vi "RenameClass.vi"(0 "ClassWriterNative.lvclass":refnum<class "ClassWriterNative.lvclass">, 1 "ClassRef":refnum<vi>, 2 "NewClassPath":path, 4 "RelinkWholeProject":bool, 5 "error in (no error)":errorcluster) -> (14 "ClassWriterNative.lvclass":refnum<class "ClassWriterNative.lvclass">, 19 "error out":errorcluster={"status"=TRUE, "code"=1026, "source"="Invoke Node in ClassWriterGOOP300.lvclass:RenameClass.vi"})   [LabVIEW 2020, in "ClassWriterNative.lvclass"]
uses:
  ClassWriterNative.lvclass
  f5b91c3c-2b4b-4460-aca0-bdbd4ce9a051.vi
  313d9ab2-2167-4cbd-8752-784b5e159654.vi
  a4843f61-b178-4b78-a5e8-dfb32b4ec01f.vi
  Common/ScriptingFunctions/Scripting.lvclass
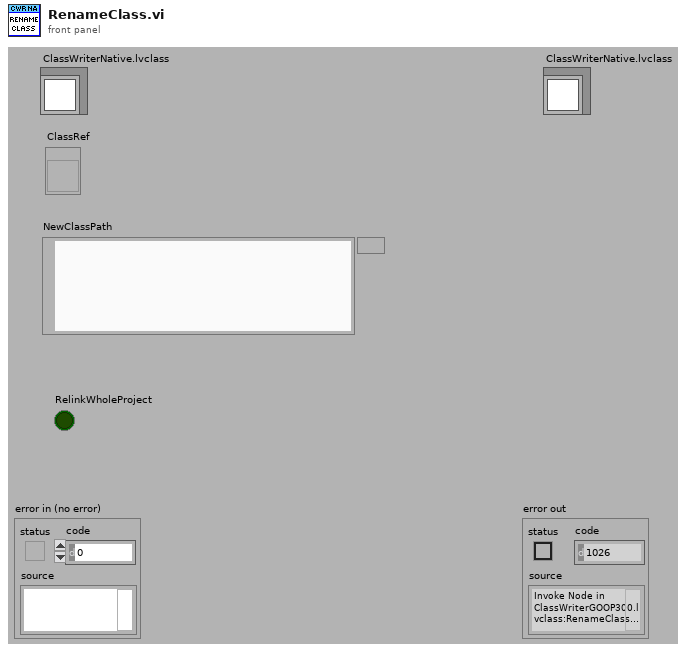
[diagram p1: front panel]
types:
  T1 = cluster{"SubClass":bool, "ClassFiles":path[], "ClassName":string, "ClassFolder":path, "VIs":refnum<vi>[], "TemplateFolder":path, "ViSubDirs":string[], "TemplateName":string, "BaseClassFolder":path, "TemplateClasses":refnum<vi>[], "Application":refnum<vi>}
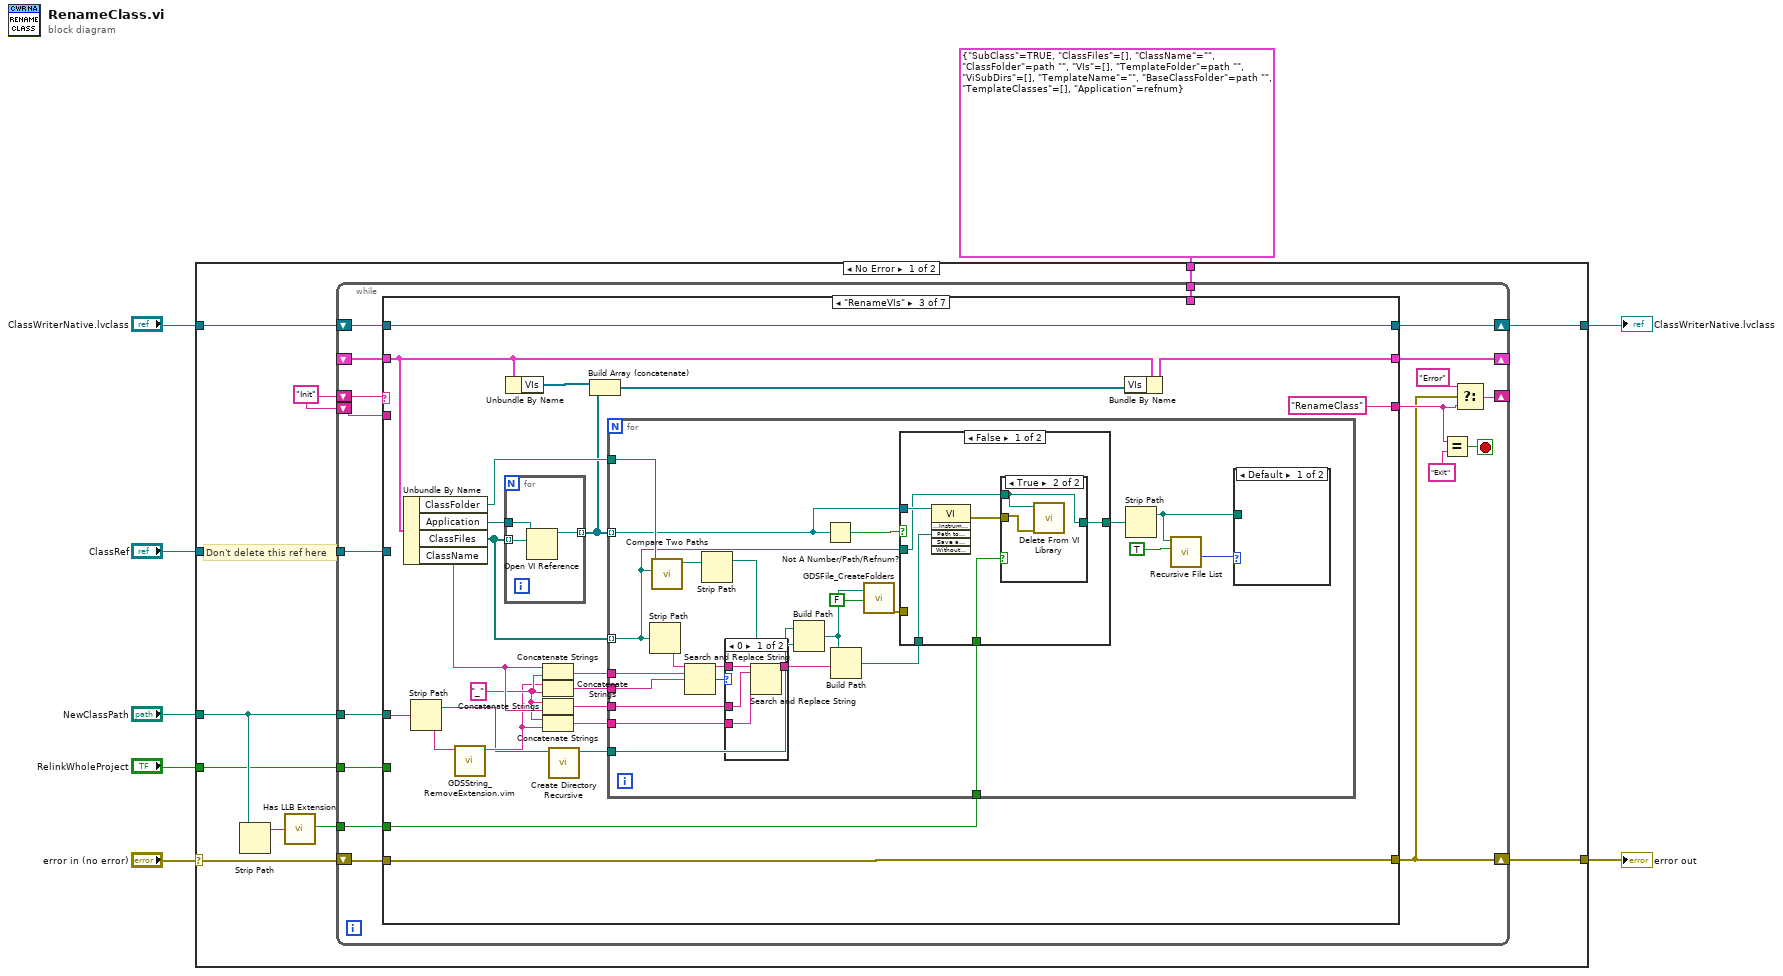
[diagram p0: block diagram]
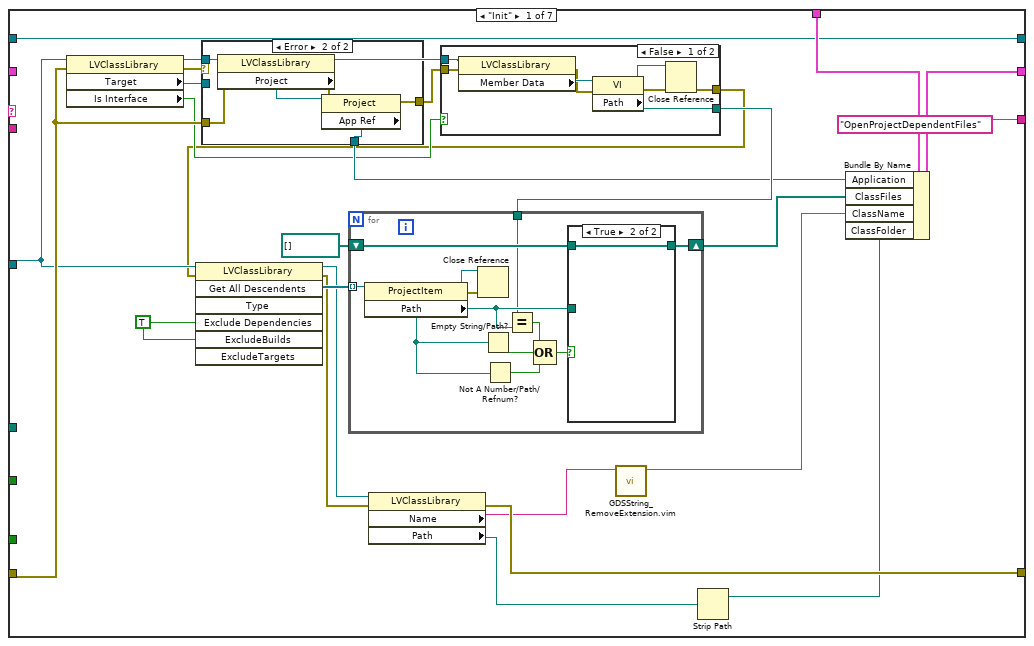
[diagram p2: hidden frame]
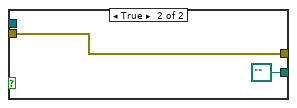
[diagram p3: hidden frame]
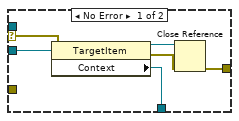
[diagram p4: hidden frame]
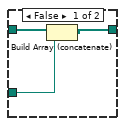
[diagram p5: hidden frame]
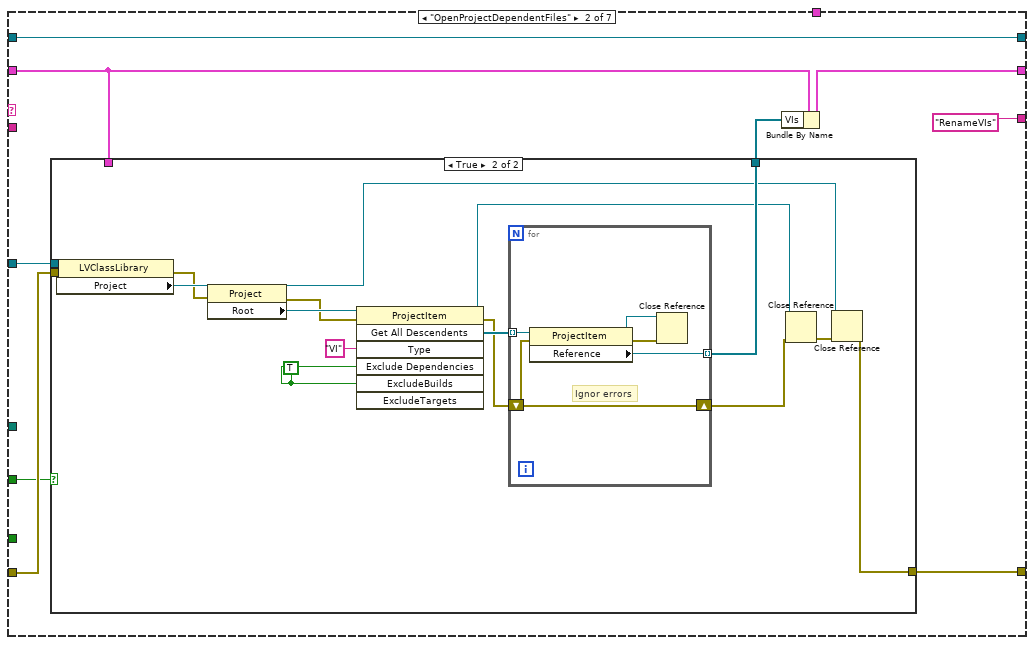
[diagram p6: hidden frame]
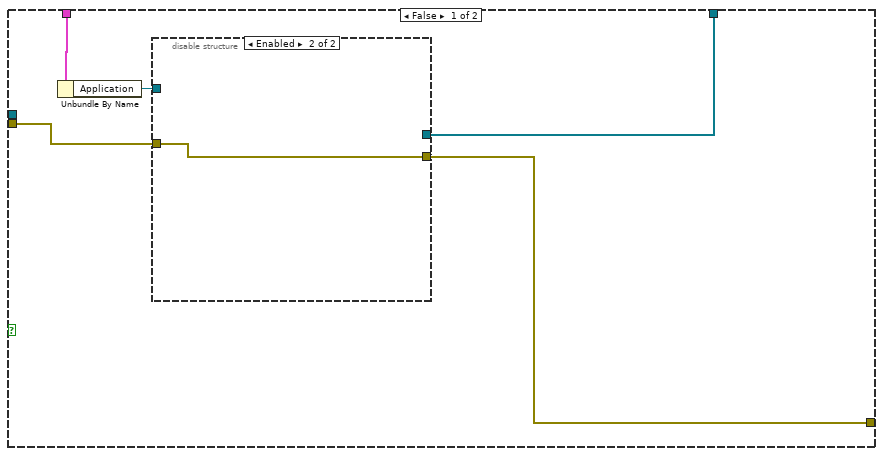
[diagram p7: hidden frame]
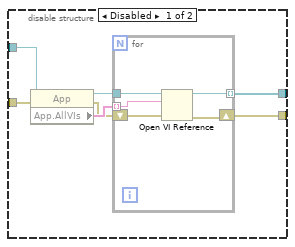
[diagram p8: hidden frame]
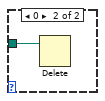
[diagram p10: hidden frame]
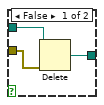
[diagram p11: hidden frame]
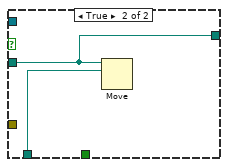
[diagram p12: hidden frame]
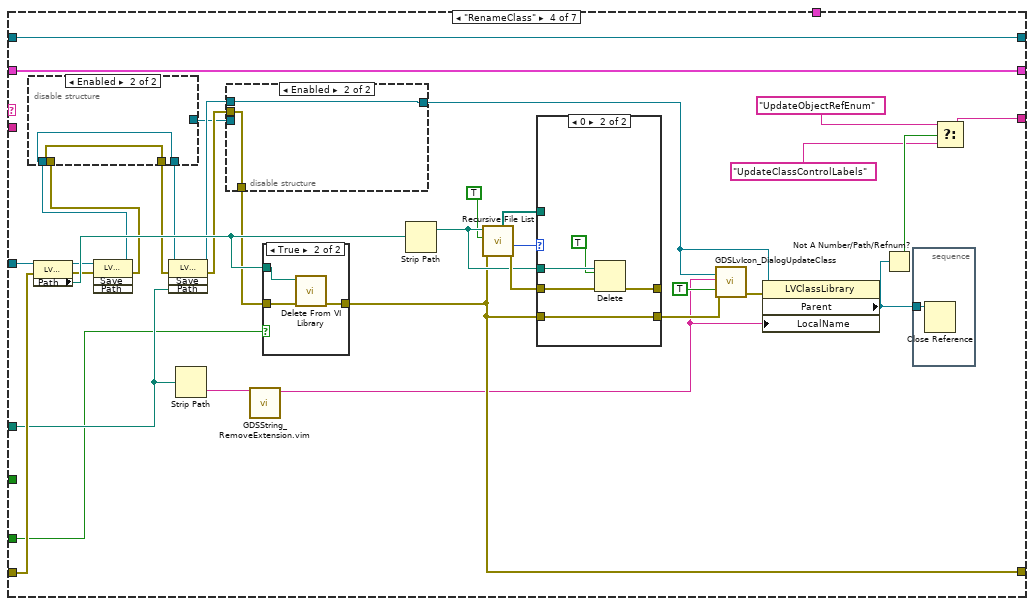
[diagram p13: hidden frame]
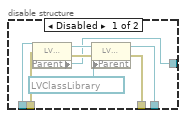
[diagram p14: hidden frame]
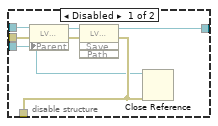
[diagram p15: hidden frame]
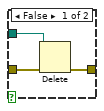
[diagram p16: hidden frame]
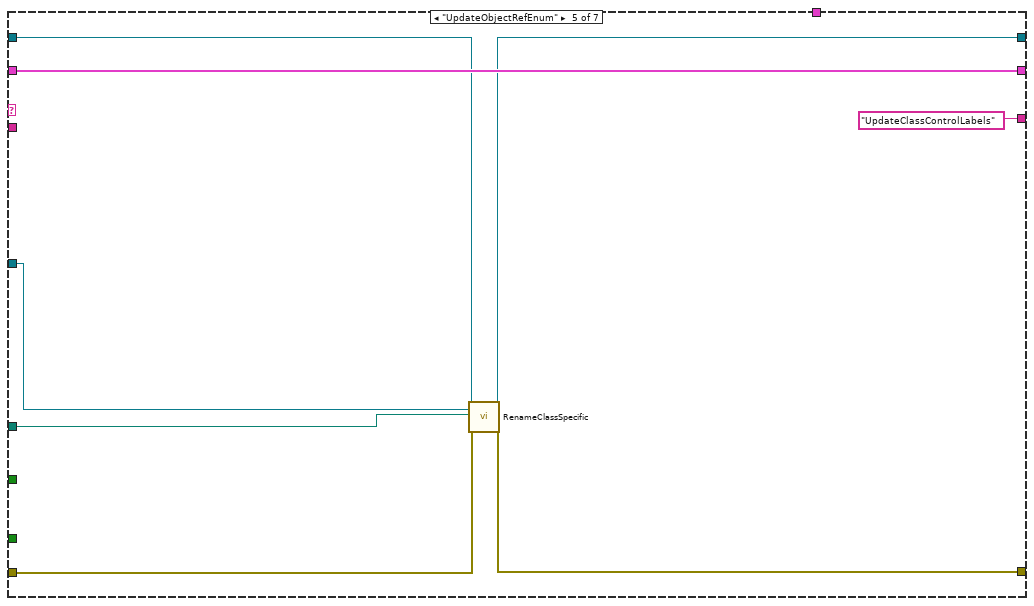
[diagram p18: hidden frame]
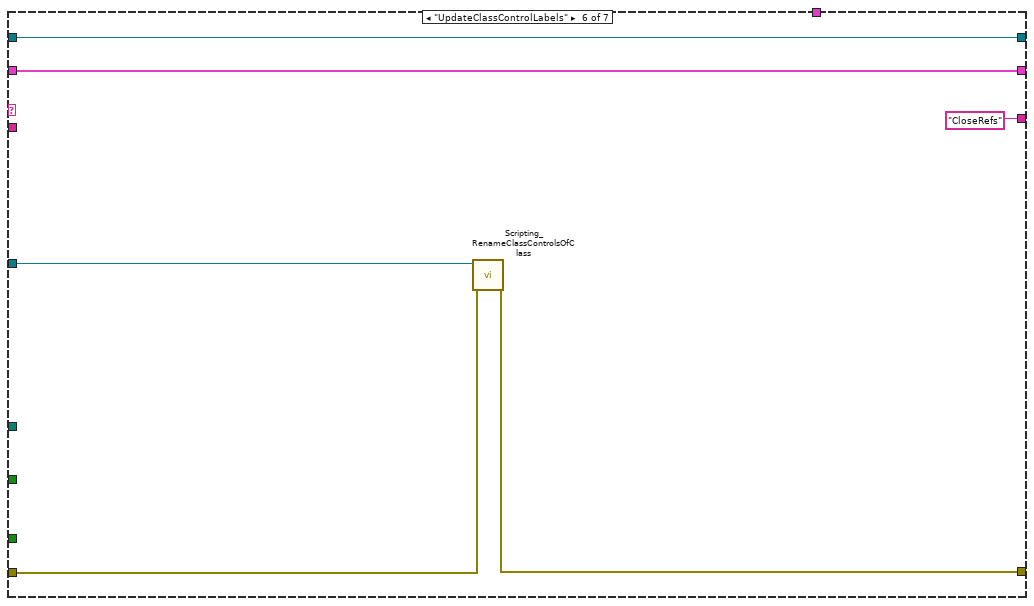
[diagram p19: hidden frame]
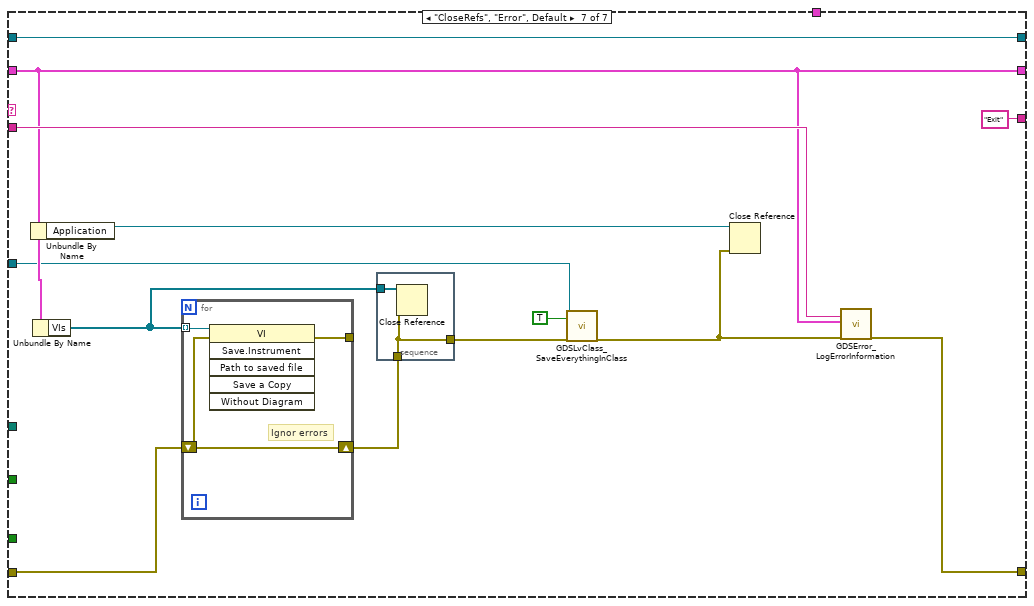
[diagram p20: hidden frame]
diagram:
  n1 = case shown="No Error" "error in (no error)" {
    selector: "error in (no error)" -> [w18 w317]
    tunnel: [w17 w317] -> w8
    tunnel: "ClassRef" -> [w19 _]
    tunnel: T1 {"SubClass"=TRUE, "ClassFiles"=[], "ClassName"="", "ClassFolder"=path "", "VIs"=[], "TemplateFolder"=path "", "ViSubDirs"=[], "TemplateName"="", "BaseClassFolder"=path "", "TemplateClasses"=[], "Application"=refnum} ("output cluster") -> [w16 _]
    tunnel: "NewClassPath" -> [w12 _]
    tunnel: "ClassWriterNative.lvclass" -> [w14 w316]
    tunnel: [w13 w316] -> w2
    tunnel: "RelinkWholeProject" -> [w9 _]
    frame No Error {
      w15 = "Init"
      # "Don't delete this ref here"
      n2 = Strip Path(path=w12) -> (stripped path=w10:path)  [unwired: 1 out]
      n3 = call <vilib>:"Has LLB Extension.vi"("path"=w10) -> ("path to VI library?"=w11:bool)
      n4 = while {
        tunnel: w19 -> [w37]
        shift-right: [w26] -> w17
        shift-left: w18 -> [w36]
        shift-right: [w31] -> _
        shift-left: w15 -> [w27]
        shift-right: [w34] -> _
        shift-left: _ -> [w35]
        tunnel: w16 -> [w29]
        tunnel: w12 -> [w25]
        shift-left: w15 -> [w24]
        shift-right: [w22] -> w13
        shift-left: w14 -> [w23]
        tunnel: w11 -> [w21]
        tunnel: w9 -> [w20]
        stop <- w32 stop-if-true
        n5 = case shown="\"RenameVIs\"" w27 {
          tunnel: w35 -> [_ w100 w163 w250 w290 w296 w305]
          tunnel: [w61 w105 w164 w250 w290 w296 w305] -> w34
          tunnel: w37 -> [w44 w107 _ w249 w289 w292 w302]
          tunnel: w36 -> [w45 w106 w169 w248 w287 w294 w309]
          tunnel: [w54 w103 w169 w220 w286 w293 w307] -> w26
          tunnel: ["OpenProjectDependentFiles" "RenameVIs" "RenameClass" w242 "UpdateClassControlLabels" "CloseRefs" "Exit"] -> w28
          tunnel: w29 -> [w60 _ _ _ _ _ _]
          tunnel: w25 -> [_ _ w167 w246 w288 _ _]
          tunnel: w24 -> [_ _ _ _ _ _ w306]
          tunnel: w23 -> [w48 w102 w158 w239 w285 w295 w304]
          tunnel: [w48 w102 w158 w239 w284 w295 w304] -> w22
          tunnel: w21 -> [_ _ w152 w232 _ _ _]
          tunnel: w20 -> [_ w101 _ _ _ _ _]
          frame "Init" {
            w47 = TRUE ("ExcludeDependencies")
            n6 = property class="LVClassLibrary"(reference=w44, error in=w45) -> (reference out=w38:refnum<vi>, error out=w46:errorcluster, "Target"=w50:refnum<vi>, "Is Interface"=w43:bool)
            n7 = case shown="Error" w46 {
              selector: w46 -> [w73 _]
              tunnel: w50 -> [w78 _]
              tunnel: [w75 w81] -> w42
              tunnel: [w74 w82] -> w49
              tunnel: w38 -> [_ w84]
              tunnel: w45 -> [_ w79]
              frame No Error {
                n8 = property class="TargetItem"(reference=w78, error in=w73) -> (reference out=w76:refnum<vi>, error out=w77:errorcluster, "Context"=w74:refnum<vi>)
                n9 = Close Reference(reference=w76, error in (no error)=w77) -> (error out=w75:errorcluster)
              }
              frame Error {
                n10 = property class="LVClassLibrary"(reference=w84, error in=w79) -> (error out=w80:errorcluster, "Project"=w83:refnum<vi>)  [unwired: 1 out]
                n11 = property class="Project"(reference=w83, error in=w80) -> (error out=w81:errorcluster, "App Ref"=w82:refnum<vi>)  [unwired: 1 out]
              }
            }
            n12 = case shown="False" w43 {
              tunnel: [w68 path "" ("Path")] -> w51
              tunnel: w42 -> [w66 w72]
              tunnel: [w64 w72] -> w41
              tunnel: w38 -> [w63 _]
              frame False {
                n13 = property class="LVClassLibrary"(reference=w63, error in=w66) -> (error out=w65:errorcluster, "Member Data"=w67:refnum<vi>)  [unwired: 1 out]
                n14 = property class="VI"(reference=w67, error in=w65) -> (reference out=w69:refnum<vi>, error out=w70:errorcluster, "Path"=w68:path)
                n15 = Close Reference(reference=w69, error in (no error)=w70) -> (error out=w64:errorcluster)
              }
              frame True {
              }
            }
            n16 = invoke class="LVClassLibrary" method="Get All Descendents"(reference=w44, error in=w41, "Exclude Dependencies"=w47, "ExcludeBuilds"=w47) -> (reference out=w56:refnum<vi>, error out=w55:errorcluster, "All Descendents"=w59:refnum<vi>[])  [unwired: 3 in, 4 out]
            n17 = for {
              tunnel: w59 -> [w91] mode=indexing
              shift-right: [w94] -> w57
              shift-left: path[] [] -> [w95]
              tunnel: w51 -> [w89]
              n18 = property class="ProjectItem"(reference=w91) -> (reference out=w93:refnum<vi>, error out=w92:errorcluster, "Path"=w90:path)  [unwired: 1 in]
              n19 = Close Reference(reference=w93, error in (no error)=w92) -> ()  [unwired: 1 out]
              n20 = Empty String/Path?(string/path=w90) -> (empty?=w87:bool)
              n21 = Not A Number/Path/Refnum?(number/path/refnum=w90) -> (NaN/Path/Refnum?=w88:bool)
              n22 = Equal?(x=w89, y=w90) -> (x = y?=w86:bool)
              n23 = Compound Arithmetic op=OR(w86, w87, w88) -> (w85:bool)
              n24 = case shown="True" w85 {
                tunnel: w95 -> [w98 w99]
                tunnel: w90 -> [w97 _]
                tunnel: [w96 w99] -> w94
                frame False {
                  n25 = Build Array (concatenate)(w98, w97) -> (w96:path[])
                }
                frame True {
                }
              }
            }
            n26 = property class="LVClassLibrary"(reference=w56, error in=w55) -> (error out=w54:errorcluster, "Name"=w40:string, "Path"=w53:path)  [unwired: 1 out]
            n27 = call "GDSString_RemoveExtension.vim"("NameWithExtension"=w40) -> ("NameWithoutExtension"=w39:string)  [unwired: 9 in, 1 out]
            n28 = Strip Path(path=w53) -> (stripped path=w52:path)  [unwired: 1 out]
            n29 = Bundle By Name(cluster=w60, "Application"=w49, "ClassFiles"=w57, "ClassName"=w39, "ClassFolder"=w52) -> (w61:T1)
          }
          frame "OpenProjectDependentFiles" {
            n30 = case shown="True" w101 {
              tunnel: w107 -> [_ w142]
              tunnel: w106 -> [w109 w137]
              tunnel: [w113 w134] -> w104
              tunnel: [w112 w128] -> w103
              tunnel: w100 -> [w111 _]
              frame False {
                n31 = Unbundle By Name(w111) -> ("Application"=w110:refnum<vi>)
                n32 = disable-structure shown="Enabled" {
                  disable-tunnel: [w117 _] -> w113
                  disable-tunnel: [w116 w126] -> w112
                  disable-tunnel: w110 -> [w115 _]
                  disable-tunnel: w109 -> [w114 w126]
                  frame Disabled {
                    n33 = property class="App"(reference=w115, error in=w114) -> (reference out=w120:refnum<vi>, error out=w118:errorcluster, "App.AllVIs"=w119:string[])
                    n34 = for {
                      tunnel: w120 -> [w125]
                      tunnel: w119 -> [w124] mode=indexing
                      shift-right: [w122] -> w116
                      shift-left: w118 -> [w123]
                      tunnel: [w121] -> w117 mode=indexing
                      n35 = Open VI Reference(application reference (local)=w125, vi path=w124, error in (no error)=w123) -> (vi reference=w121:refnum<vi>, error out=w122:errorcluster)  [unwired: 3 in]
                    }
                  }
                  frame Enabled {
                  }
                }
              }
              frame True {
                w127 = TRUE ("ExcludeDependencies")
                n36 = property class="LVClassLibrary"(reference=w142, error in=w137) -> (error out=w138:errorcluster, "Project"=w141:refnum<vi>)  [unwired: 1 out]
                n37 = property class="Project"(reference=w141, error in=w138) -> (reference out=w129:refnum<vi>, error out=w136:errorcluster, "Root"=w140:refnum<vi>)
                n38 = invoke class="ProjectItem" method="Get All Descendents"(reference=w140, error in=w136, "Type"="VI", "Exclude Dependencies"=w127, "ExcludeBuilds"=w127) -> (reference out=w131:refnum<vi>, error out=w133:errorcluster, "All Descendents"=w135:refnum<vi>[])  [unwired: 2 in, 4 out]
                n39 = for {
                  tunnel: w135 -> [w147] mode=indexing
                  tunnel: [w146] -> w134 mode=indexing
                  shift-right: [w143] -> w132
                  shift-left: w133 -> [w143]
                  # "Ignor errors"
                  n40 = property class="ProjectItem"(reference=w147, error in=w143) -> (reference out=w144:refnum<vi>, error out=w145:errorcluster, "Reference"=w146:refnum<vi>)
                  n41 = Close Reference(reference=w144, error in (no error)=w145) -> ()  [unwired: 1 out]
                }
                n42 = Close Reference(reference=w131, error in (no error)=w132) -> (error out=w130:errorcluster)
                n43 = Close Reference(reference=w129, error in (no error)=w130) -> (error out=w128:errorcluster)
              }
            }
            n44 = Bundle By Name(cluster=w100, "VIs"=w104) -> (w105:T1)
          }
          frame "RenameVIs" {
            w155 = "_" ("string")
            n45 = Unbundle By Name(w163) -> ("ClassFolder"=w165:path, "Application"=w159:refnum<vi>, "ClassFiles"=w168:path[], "ClassName"=w156:string)
            n46 = Strip Path(path=w167) -> (stripped path=w148:path, name=w151:string)
            n47 = call "GDSString_RemoveExtension.vim"("NameWithExtension"=w151) -> ("NameWithoutExtension"=w150:string)  [unwired: 9 in, 1 out]
            n48 = for {
              tunnel: w168 -> [w216] mode=indexing
              tunnel: [w215] -> w161 mode=indexing
              tunnel: w159 -> [w214]
              n49 = Open VI Reference(application reference (local)=w214, vi path=w216) -> (vi reference=w215:refnum<vi>)  [unwired: 4 in, 1 out]
            }
            n50 = Unbundle By Name(w163) -> ("VIs"=w162:refnum<vi>[])
            n51 = Concatenate Strings(w156, w155) -> (w157:string)
            n52 = Concatenate Strings(w150, w155) -> (w166:string)
            n53 = Concatenate Strings(w155, w156) -> (w154:string)
            n54 = Concatenate Strings(w155, w150) -> (w153:string)
            n55 = call <vilib>:"Create Directory Recursive.vi"("directory"=w148) -> ("directory copy"=w149:path)  [unwired: 4 in, 2 out]
            n56 = Build Array (concatenate)(w162, w161) -> (w160:refnum<vi>[])
            n57 = for {
              tunnel: w161 -> [w180] mode=indexing
              tunnel: w168 -> [w183] mode=indexing
              tunnel: w157 -> [w194]
              tunnel: w166 -> [w193]
              tunnel: w149 -> [w192]
              tunnel: w165 -> [w191]
              tunnel: w154 -> [w177]
              tunnel: w153 -> [w176]
              tunnel: w152 -> [w175]
              n58 = Strip Path(path=w183) -> (name=w190:string)  [unwired: 1 out]
              n59 = call <vilib>:"Compare Two Paths.vi"("Path 2"=w183, "Path 1"=w191) -> ("Relative Path from 1 to 2"=w189:path)  [unwired: 6 in, 3 out]
              n60 = Search and Replace String(input string=w190, search string=w194, replace string=w193) -> (result string=w179:string, number of replacements=w171:i32)  [unwired: 5 in, 2 out]
              n61 = Strip Path(path=w189) -> (stripped path=w188:path)  [unwired: 1 out]
              n62 = case shown="0" w171 {
                tunnel: w179 -> [w198 w199]
                tunnel: [w197 w199] -> w178
                tunnel: w177 -> [w196 _]
                tunnel: w176 -> [w195 _]
                frame 0 {
                  n63 = Search and Replace String(input string=w198, search string=w196, replace string=w195) -> (result string=w197:string)  [unwired: 5 in, 3 out]
                }
                frame Default {
                }
              }
              n64 = Build Path(base path=w192, name or relative path=w188) -> (appended path=w187:path)
              n65 = Not A Number/Path/Refnum?(number/path/refnum=w180) -> (NaN/Path/Refnum?=w185:bool)
              n66 = Build Path(base path=w187, name or relative path=w178) -> (appended path=w182:path)
              n67 = call "GDSFile_CreateFolders.vi"("Path"=w187, "Promt if folder\ndoes not exists?"=FALSE ("Promt if folder\ndoes not exists?")) -> ("error out"=w184:errorcluster)  [unwired: 13 in, 4 out]
              n68 = case shown="False" w185 {
                tunnel: w184 -> [_ _]
                tunnel: w183 -> [w202 w212]
                tunnel: w182 -> [w205 w213]
                tunnel: [w204 w212] -> w181
                tunnel: w180 -> [w206 _]
                tunnel: w175 -> [w201 _]
                frame False {
                  n69 = invoke class="VI" method="Save.Instrument"(reference=w206, "Path to saved file"=w205) -> (error out=w203:errorcluster)  [unwired: 4 in, 5 out]
                  n70 = case shown="True" w201 {
                    tunnel: [w209 w211] -> w204
                    tunnel: w203 -> [w208 w210]
                    tunnel: w202 -> [w207 w211]
                    frame False {
                      n71 = Delete(path (use dialog)=w207, error in=w208) -> (deleted path=w209:path)  [unwired: 3 in, 2 out]
                    }
                    frame True {
                      n72 = call <vilib>:"Delete From VI Library.vi"("error in (no error)"=w210, "path"=w211) -> ()  [unwired: 9 in, 1 out]
                    }
                  }
                }
                frame True {
                  n73 = Move(source path=w212, 10:w213) -> ()  [unwired: 3 in, 3 out]
                }
              }
              n74 = Strip Path(path=w181) -> (stripped path=w173:path)  [unwired: 1 out]
              n75 = call <vilib>:"Recursive File List.vi"("Treat LLBs as Folders?"=TRUE, "Folder Path"=w173) -> ("Number of Files"=w172:i32)  [unwired: 5 in, 4 out]
              n76 = case shown="Default" w172 {
                tunnel: w173 -> [_ w200]
                frame Default {
                }
                frame 0 {
                  n77 = Delete(path (use dialog)=w200) -> ()  [unwired: 4 in, 3 out]
                }
              }
            }
            n78 = Bundle By Name(cluster=w163, "VIs"=w160) -> (w164:T1)
          }
          frame "RenameClass" {
            n79 = property class="LVClassLibrary"(reference=w249, error in=w248) -> (reference out=w231:refnum<vi>, error out=w230:errorcluster, "Path"=w233:path)
            n80 = invoke class="LVClassLibrary" method="Save"(reference=w231, error in=w230) -> (reference out=w229:refnum<vi>, error out=w228:errorcluster)  [unwired: 2 in, 2 out]
            n81 = disable-structure shown="Enabled" {
              disable-tunnel: w229 -> [w258 w260]
              disable-tunnel: w228 -> [w257 w259]
              disable-tunnel: [w253 w260] -> w227
              disable-tunnel: [w252 w259] -> w226
              disable-tunnel: [w251 _] -> w217
              frame Disabled {
                n82 = property class="LVClassLibrary"(reference=w258, error in=w257) -> (reference out=w256:refnum<vi>, error out=w255:errorcluster, "Parent"=w251:refnum<vi>)
                n83 = property class="LVClassLibrary"(reference=w256, error in=w255, "Parent"=refnum<vi> refnum ("Parent Class")) -> (reference out=w253:refnum<vi>, error out=w252:errorcluster)
              }
              frame Enabled {
              }
            }
            n84 = invoke class="LVClassLibrary" method="Save"(reference=w227, error in=w226, "Path"=w246) -> (reference out=w225:refnum<vi>, error out=w224:errorcluster)  [unwired: 1 in, 2 out]
            n85 = Strip Path(path=w246) -> (name=w219:string)  [unwired: 1 out]
            n86 = disable-structure shown="Enabled" {
              disable-tunnel: w225 -> [w267 w268]
              disable-tunnel: w224 -> [w266 w269]
              disable-tunnel: [w263 w268] -> w223
              disable-tunnel: [w262 w269] -> w222
              disable-tunnel: w217 -> [w261 _]
              frame Disabled {
                n87 = property class="LVClassLibrary"(reference=w267, error in=w266, "Parent"=w261) -> (reference out=w265:refnum<vi>, error out=w264:errorcluster)
                n88 = invoke class="LVClassLibrary" method="Save"(reference=w265, error in=w264) -> (reference out=w263:refnum<vi>, error out=w262:errorcluster)  [unwired: 2 in, 2 out]
                n89 = Close Reference(reference=w261, error in (no error)=w262) -> ()  [unwired: 1 out]
              }
              frame Enabled {
              }
            }
            n90 = call "GDSString_RemoveExtension.vim"("NameWithExtension"=w219) -> ("NameWithoutExtension"=w218:string)  [unwired: 9 in, 1 out]
            n91 = case shown="True" w232 {
              tunnel: w222 -> [w272 w273]
              tunnel: w233 -> [w271 w275]
              tunnel: [w270 w274] -> w220
              frame False {
                n92 = Delete(path (use dialog)=w271, error in=w272) -> (error out=w270:errorcluster)  [unwired: 3 in, 2 out]
              }
              frame True {
                n93 = call <vilib>:"Delete From VI Library.vi"("error in (no error)"=w273, "path"=w275) -> ("error out"=w274:errorcluster)  [unwired: 9 in]
              }
            }
            n94 = Strip Path(path=w233) -> (stripped path=w235:path)  [unwired: 1 out]
            n95 = call <vilib>:"Recursive File List.vi"("error in (no error)"=w220, "Treat LLBs as Folders?"=TRUE, "Folder Path"=w235) -> ("error out"=w237:errorcluster, "Number of Files"=w238:i32, "All Folders"=w236:path[])  [unwired: 4 in, 2 out]
            n96 = case shown="0" w238 {
              tunnel: w235 -> [_ w283]
              tunnel: w237 -> [w278 w280]
              tunnel: [w278 w281] -> _
              tunnel: w236 -> [_ _]
              tunnel: [w277 w279] -> w221
              tunnel: w220 -> [w277 w279]
              frame Default {
              }
              frame 0 {
                n97 = Delete(path (use dialog)=w283, entire hierarchy (F)=TRUE, error in=w280) -> (error out=w281:errorcluster)  [unwired: 2 in, 2 out]
              }
            }
            n98 = call "GDSLvIcon_DialogUpdateClass.vi"("ClassPath(FilePath/ProjectTreePath/LvCLassRef)"=w223, "ClassName"=w218, "AutoUpdate"=TRUE, "error in (no error)"=w221) -> ("error out"=w245:errorcluster)  [unwired: 12 in, 3 out]
            n99 = property class="LVClassLibrary"(reference=w223, error in=w245, "LocalName"=w218) -> ("Parent"=w244:refnum<vi>)  [unwired: 2 out]
            n100 = Not A Number/Path/Refnum?(number/path/refnum=w244) -> (NaN/Path/Refnum?=w243:bool)
            n101 = stacked-sequence {
              tunnel: w244 -> [w276]
              frame #0 {
                n102 = Close Reference(reference=w276) -> ()  [unwired: 1 in, 1 out]
              }
            }
            n103 = Select(t="UpdateObjectRefEnum", s=w243, f="UpdateClassControlLabels") -> (s? t:f=w242:string)
          }
          frame "UpdateObjectRefEnum" {
            n104 = call-dynamic "RenameClassSpecific.vi"("ClassWriterNative.lvclass"=w285, "ClassRef"=w289, "NewClassPath"=w288, "error in"=w287) -> ("ClassWriterNative.lvclass"=w284:refnum<class "ClassWriterNative.lvclass">, "error out"=w286:errorcluster)  [unwired: 14 in]
          }
          frame "UpdateClassControlLabels" {
            n105 = call "Scripting_RenameClassControlsOfClass.vi"("error in (no error)"=w294, "LVClassLibrary in"=w292) -> ("error out"=w293:errorcluster)  [unwired: 9 in]
          }
          frame "CloseRefs", "Error", Default {
            n106 = Unbundle By Name(w305) -> ("Application"=w308:refnum<vi>)
            n107 = Unbundle By Name(w305) -> ("VIs"=w300:refnum<vi>[])
            n108 = for {
              tunnel: w300 -> [w315] mode=indexing
              shift-right: [w314] -> w299
              shift-left: w309 -> [w314]
              tunnel: [w313] -> _
              # "Ignor errors"
              n109 = invoke class="VI" method="Save.Instrument"(reference=w315, error in=w314) -> (error out=w313:errorcluster)  [unwired: 4 in, 5 out]
            }
            n110 = stacked-sequence {
              tunnel: w300 -> [w312]
              tunnel: w299 -> [w311]
              tunnel: [w311] -> w298
              frame #0 {
                n111 = Close Reference(reference=w312, error in (no error)=w311) -> ()  [unwired: 1 out]
              }
            }
            n112 = call "GDSLvClass_SaveEverythingInClass.vi"("ClassRefIn"=w302, "ForceResaving(False)"=TRUE, "error in"=w298) -> ("error out"=w303:errorcluster)  [unwired: 15 in, 1 out]
            n113 = Close Reference(reference=w308, error in (no error)=w303) -> ()  [unwired: 1 out]
            n114 = call "GDSError_LogErrorInformation.vi"("State"=w306, "LocalVariableData"=w305, "error in (no error)"=w303) -> ("error out"=w307:errorcluster)  [unwired: 16 in]
          }
        }
        n115 = Equal?(x=w28, y="Exit") -> (x = y?=w32:bool)
        n116 = Select(t="Error", s=w26, f=w28) -> (s? t:f=w31:string)
      }
    }
    frame Error {
    }
  }
  "ClassWriterNative.lvclass" <- w2
  "error out" <- w8
